vi "_CSMOFGV Dequeue.vi"(8 "Error In":errorcluster caption="error in (no error)", 9 "Dequeue Timeout (0ms)":i32, 10 "State (S) In (\"\")":string, 11 "CSMQ In":T1={"info"={"Module Name"="", "Requested Name"="", "Group Name"="", "Mode"=enum."Stand Alone", "Allowed Messages"=[]}, "Refs"={"WatchDogQ"=refnum, "CSMDataDVR"=refnum, "Queue"={"HPriorityQ"=refnum, "LowPriorityQ"=refnum}, "GroupDataDVR"=refnum, "TagMap"=refnum, "ExitEvent"=refnum, "NewStateEvent"=refnum, "StatusEvent"=refnum, "InterruptEvent"=refnum}}) -> (0 "error out":errorcluster, 2 "States Out":string, 3 "CSMQ Out":T1={"info"={"Module Name"="", "Requested Name"="", "Group Name"="", "Mode"=enum."Stand Alone", "Allowed Messages"=[]}, "Refs"={"WatchDogQ"=refnum, "CSMDataDVR"=refnum, "Queue"={"HPriorityQ"=refnum, "LowPriorityQ"=refnum}, "GroupDataDVR"=refnum, "TagMap"=refnum, "ExitEvent"=refnum, "NewStateEvent"=refnum, "StatusEvent"=refnum, "InterruptEvent"=refnum}})   [LabVIEW 2017, in "Communicable State Machine.lvlib"]
uses:
  Communicable State Machine.lvlib
  _CSMObj.ctl
  _CSMObj-Info.ctl
  Typedef/_CSM_MODE.ctl
  _CSMObj-Refs.ctl
  _CSMObj-Data.ctl
  Typedef/_CSM_MSG_TYPE.ctl
  Priority Queue/Priority Queue.ctl
  Typedef/_Cross CSM State Data.ctl
  Typedef/_Cross CSM State Response.ctl
  Typedef/_CSM_Response Source Message.ctl
  Priority Queue/def-Data(LowPRI-Q).ctl
  _CSMObj-ModeData.ctl
  Typedef/_CSM Status Change Event Data.ctl
  AdvanceAPI/CSM - Make String Arguments Safe.vi
  AdvanceAPI/CSM - Keywords.vi
  _Shared/CSM Shared.lvlib
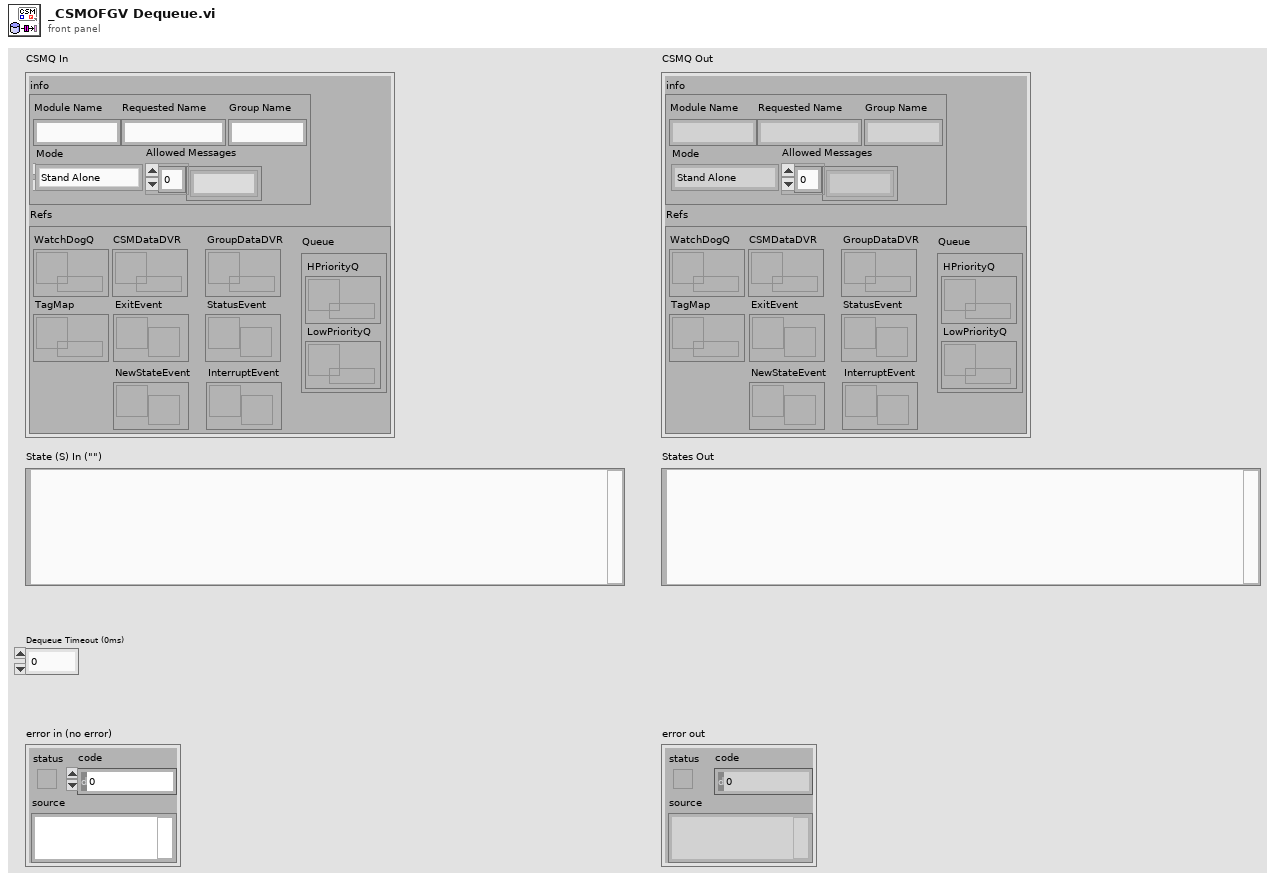
[diagram p1: front panel]
types:
  T1 = typedef "Communicable State Machine.lvlib/_CSMObj.ctl" = cluster{"info":T2, "Refs":T4}
  T2 = typedef "Communicable State Machine.lvlib/_CSMObj-Info.ctl" = cluster{"Module Name":string, "Requested Name":string, "Group Name":string, "Mode":T3, "Allowed Messages":string[]}
  T3 = typedef "Communicable State Machine.lvlib/_CSM_MODE.ctl" = enum16{"Not Exist", "Stand Alone", "CSM", "Worker", "Worker Agent", "Chain Node", "Chain"}
  T4 = typedef "Communicable State Machine.lvlib/_CSMObj-Refs.ctl" = cluster{"WatchDogQ":refnum<queue>, "CSMDataDVR":refnum<data-value>, "Queue":T5, "GroupDataDVR":refnum<data-value>, "TagMap":refnum<data-value>, "ExitEvent":refnum<user-event>, "NewStateEvent":refnum<user-event>, "StatusEvent":refnum<user-event>, "InterruptEvent":refnum<user-event>}
  T5 = typedef "Communicable State Machine.lvlib/Priority Queue.ctl" = cluster{"HPriorityQ":refnum<queue>, "LowPriorityQ":refnum<queue>}
  T6 = typedef "Communicable State Machine.lvlib/_CSM_MSG_TYPE.ctl" = enum16{"Sync Message(-@)", "Async Message(->)", "Async without Response(->|)", "Async Response", "Broadcast(-><all>)", "Broadcast(-><status>)", "Broadcast(-><interrupt>)", "Append to JKISM States", "Append to JKISM States(High Priority)", "Broadcast(-><state>)", "<None>"}
  T7 = typedef "Communicable State Machine.lvlib/_CSMObj-Data.ctl" = cluster{"RemoteMessge?":bool, "error":errorcluster, "Return State":string, "Initialized":enum16{"Initializing", "Ready", "Exiting"}, "InternalRegistryRules":string[], "Return Msg Type":T6, "Current State":string, "Remaing JKISM Queue":string}
  T8 = typedef "Communicable State Machine.lvlib/_Cross CSM State Data.ctl" = cluster{"Msg Type":T6, "state":string, "args":string, "source":string, "RespQ":refnum<queue>, "Response For Message":T9, "Target":string}
  T9 = typedef "Communicable State Machine.lvlib/_CSM_Response Source Message.ctl" = cluster{"‘State":string, "’Arguments":string, "’Error":errorcluster}
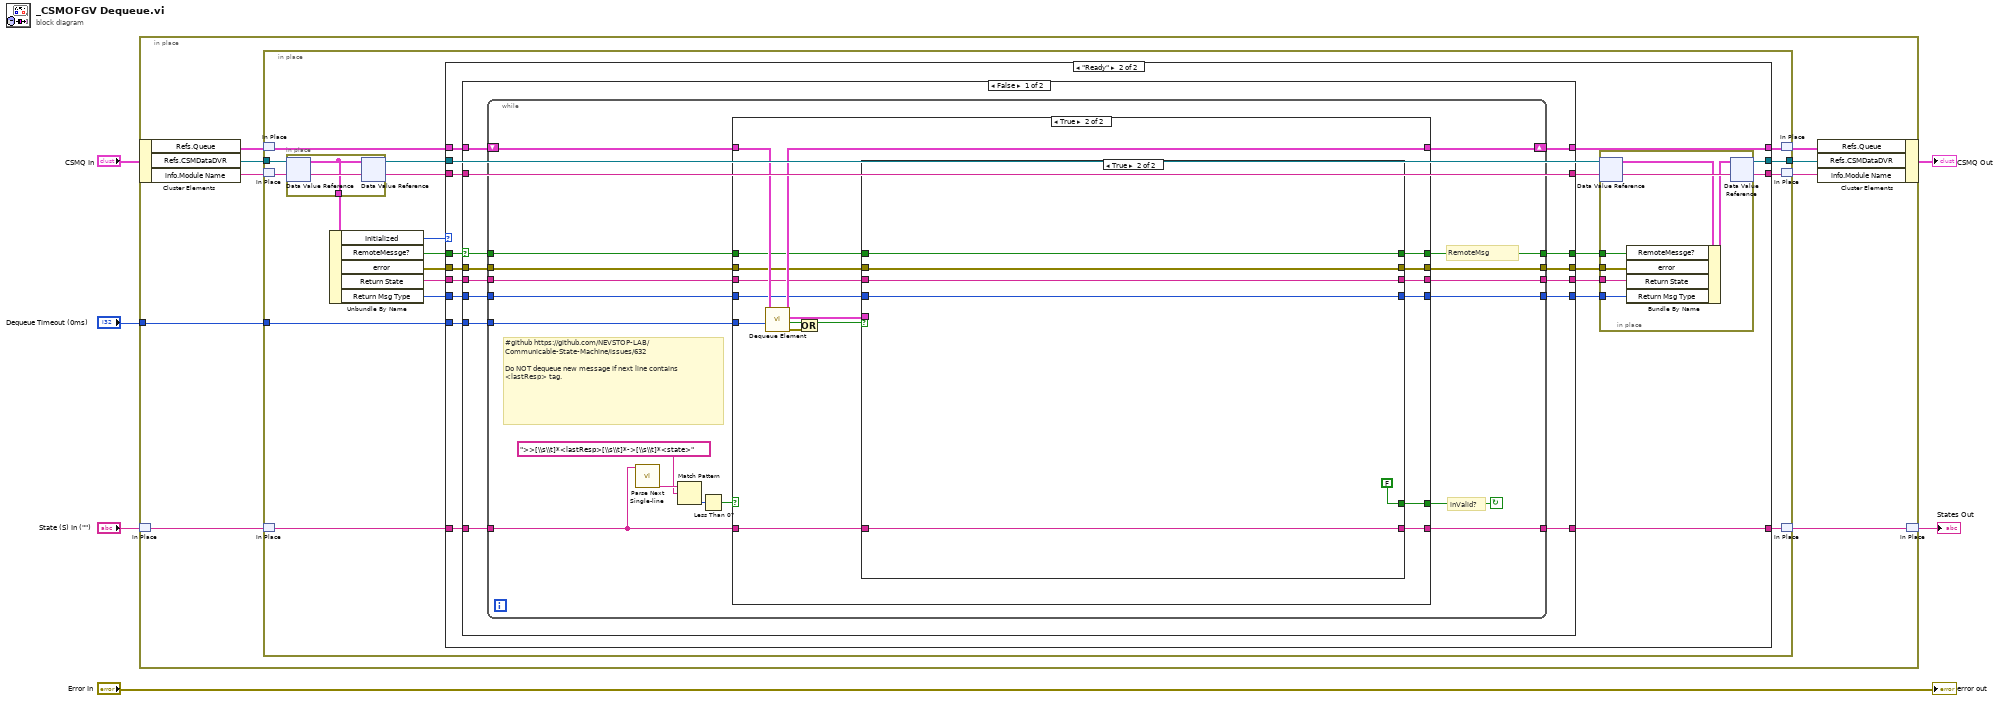
[diagram p0: block diagram]
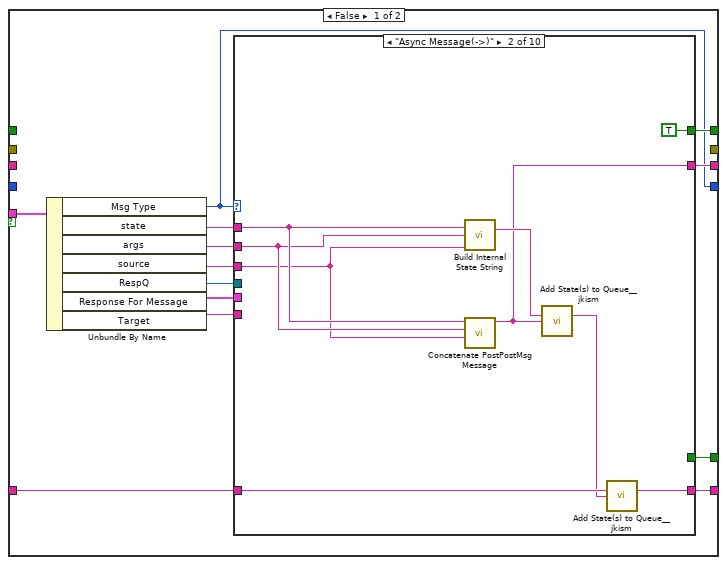
[diagram p4: hidden frame]
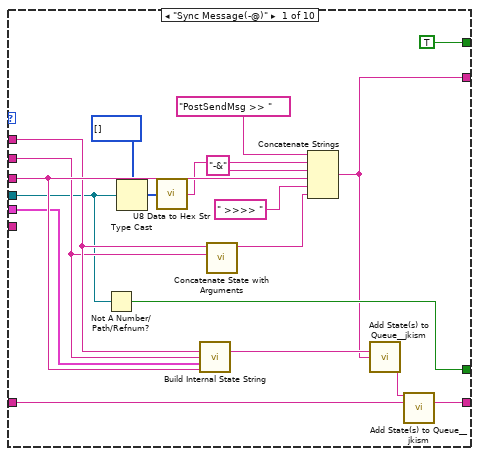
[diagram p5: hidden frame]
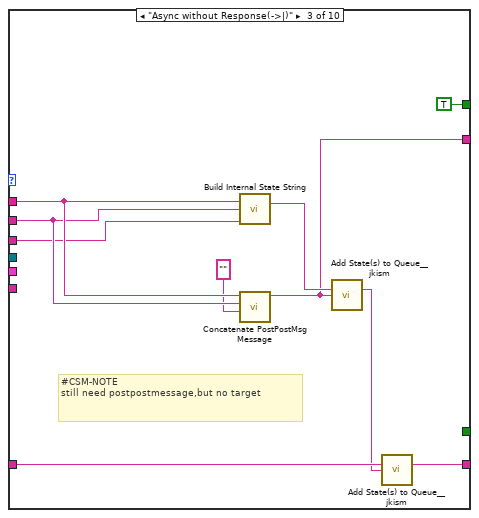
[diagram p6: hidden frame]
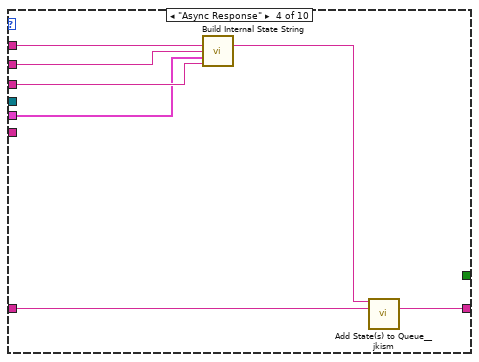
[diagram p7: hidden frame]
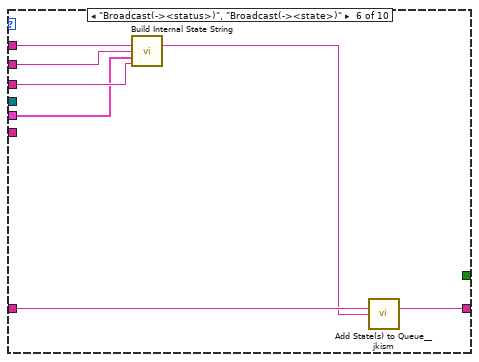
[diagram p9: hidden frame]
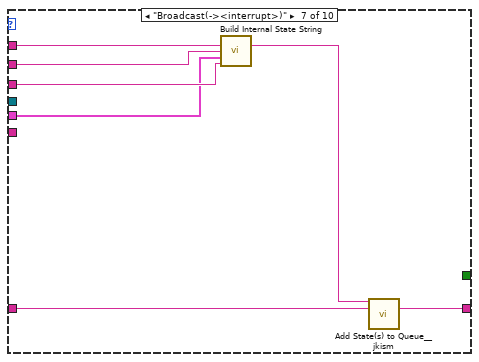
[diagram p10: hidden frame]
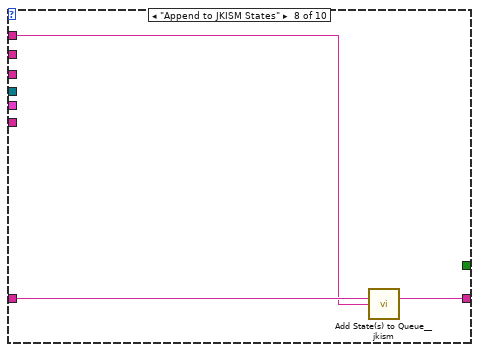
[diagram p11: hidden frame]
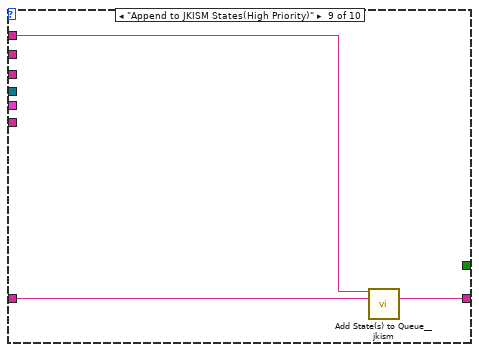
[diagram p12: hidden frame]
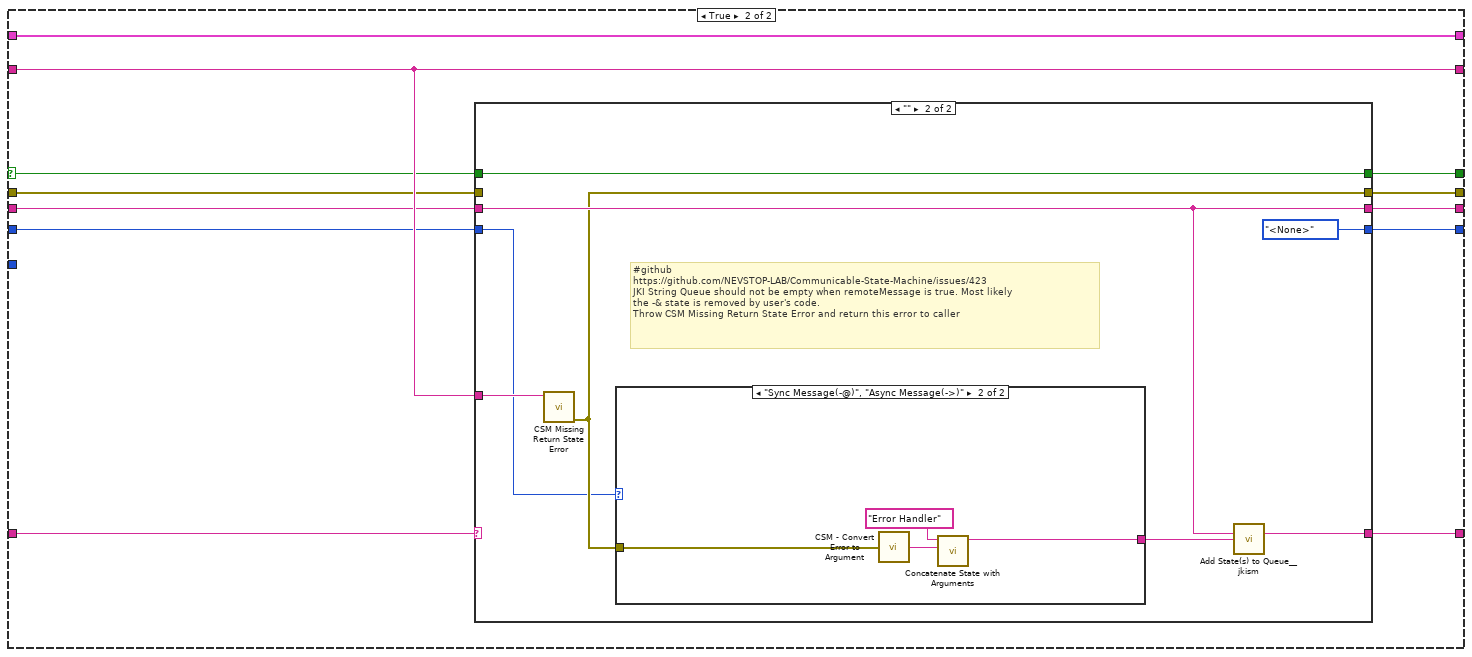
[diagram p14: hidden frame]
diagram:
  n1 = in-place "In Place Element Structure" {
    in-place-border: "Dequeue Timeout (0ms)" -> [w13]
    n2 = in-place-cluster #1("CSMQ In") -> ("Refs.Queue"=w15:T5, "Refs.CSMDataDVR"=w10:refnum<data-value>, "info.Module Name"=w7:string)
    n3 = in-place-match #2("State (S) In (\"\")") -> (w12:string)
    n4 = in-place {
      in-place-border: w13 -> [w29]
      in-place-border: w10 -> [w26]
      in-place-border: [w23] -> w9
      n5 = in-place-match #3(w15) -> (w30:T5)
      n6 = in-place-match #4(w7) -> (w19:string)
      n7 = in-place-match #5(w12) -> (w28:string)
      n8 = in-place {
        in-place-border: [w230] -> w25
        n9 = in-place-dvr #6(w26) -> (w230:T7)  [unwired: 1 out]
        n10 = in-place-dvr #6(w230) -> (w24:refnum<data-value>)  [unwired: 1 out]
      }
      n11 = Unbundle By Name(w25) -> ("Initialized"=w17:enum16{"Initializing", "Ready", "Exiting"}, "RemoteMessge?"=w22:bool, "error"=w21:errorcluster, "Return State"=w20:string, "Return Msg Type"=w16:T6)
      n12 = case shown="\"Ready\"" w17 {
        tunnel: [w35 w52] -> w31
        tunnel: w30 -> [w35 w51]
        tunnel: w29 -> [_ w50]
        tunnel: w28 -> [w32 w49]
        tunnel: [w32 w48] -> w27
        tunnel: w24 -> [w34 w47]
        tunnel: [w34 w46] -> w23
        tunnel: w22 -> [_ w44]
        tunnel: w21 -> [_ w42]
        tunnel: w20 -> [_ w40]
        tunnel: w19 -> [w33 w39]
        tunnel: [w33 w38] -> w18
        tunnel: w16 -> [_ w36]
        frame "Initializing", "Exiting", Default {
        }
        frame "Ready" {
          n13 = case shown="False" w44 {
            selector: w44 -> [w66 w203]
            tunnel: [w71 w212] -> w52
            tunnel: w51 -> [w72 w212]
            tunnel: w50 -> [w70 _]
            tunnel: w49 -> [w69 w206]
            tunnel: [w68 w205] -> w48
            tunnel: [w67 w204] -> w45
            tunnel: [w65 w210] -> w43
            tunnel: w42 -> [w64 w209]
            tunnel: [w63 w208] -> w41
            tunnel: w40 -> [w62 w207]
            tunnel: w39 -> [w61 w211]
            tunnel: [w61 w211] -> w38
            tunnel: [w60 w202] -> w37
            tunnel: w36 -> [w59 w201]
            frame False {
              n14 = while {
                tunnel: w70 -> [w88]
                shift-right: [w89] -> w71
                shift-left: w72 -> [w90]
                tunnel: w66 -> [w85]
                tunnel: [w86] -> w67
                tunnel: w69 -> [w77]
                tunnel: [w87] -> w68
                tunnel: [w83] -> w65
                tunnel: w64 -> [w82]
                tunnel: [w81] -> w63
                tunnel: w62 -> [w80]
                tunnel: [w79] -> w60
                tunnel: w59 -> [w78]
                stop <- w84 continue-if-true
                # "#github https://github.com/NEVSTOP-LAB/Communicable-State-Machine/issues/632\n\nDo NOT dequeue new message if next line contains <lastResp> tag."
                # "inValid?"
                # "RemoteMsg"
                n15 = call "Parse Next Single-line.vi"("States Queue"=w77) -> ("Next Single-line State"=w76:string)  [unwired: 9 in, 1 out]
                n16 = Match Pattern(string=w76, regular expression=">>[\\s\\t]*<lastResp>[\\s\\t]*->[\\s\\t]*<state>" ("string")) -> (offset past match=w75:i32)  [unwired: 1 in, 3 out]
                n17 = Less Than 0?(x=w75) -> (x < 0?=w74:bool)
                n18 = case shown="True" w74 {
                  tunnel: w90 -> [w96 w114]
                  tunnel: [w96 w113] -> w89
                  tunnel: w88 -> [_ w112]
                  tunnel: w77 -> [w91 w110]
                  tunnel: [w91 w109] -> w87
                  tunnel: [w94 w105] -> w86
                  tunnel: w85 -> [w94 w104]
                  tunnel: [_ w103] -> w84
                  tunnel: [w95 w102] -> w83
                  tunnel: w82 -> [w95 w101]
                  tunnel: [w93 w100] -> w81
                  tunnel: w80 -> [w93 w99]
                  tunnel: [w92 w98] -> w79
                  tunnel: w78 -> [w92 w97]
                  frame False {
                  }
                  frame True {
                    n19 = call "Dequeue Element.vi"("Timeout In ms (-1)"=w112, "Priority Queue"=w114) -> ("error out"=w106:errorcluster, "Timed Out?"=w107:bool, "Cross JKI State Machine State"=w111:T8, "Priority Queue (Dup)"=w113:T5)  [unwired: 5 in, 1 out]
                    n20 = Or(x=w107, y=w106) -> (x .or. y?=w108:bool)
                    n21 = case shown="True" w108 {
                      tunnel: w110 -> [w127 w200]
                      tunnel: [w126 w200] -> w109
                      tunnel: w111 -> [w121 _]
                      tunnel: [w118 w199] -> w105
                      tunnel: w104 -> [_ w199]
                      tunnel: [w117 FALSE] -> w103
                      tunnel: [_ w197] -> w102
                      tunnel: w101 -> [_ w197]
                      tunnel: [w116 w196] -> w100
                      tunnel: w99 -> [_ w196]
                      tunnel: [w115 w195] -> w98
                      tunnel: w97 -> [_ w195]
                      frame False {
                        n22 = Unbundle By Name(w121) -> ("Msg Type"=w115:T6, "state"=w124:string, "args"=w123:string, "source"=w122:string, "RespQ"=w125:refnum<queue>, "Response For Message"=w120:T9, "Target"=w119:string)
                        n23 = case shown="\"Async Message(->)\"" w115 {
                          tunnel: w127 -> [w146 w155 w165 w172 w173 w180 w187 w190 w193 w194]
                          tunnel: [w145 w154 w164 w171 w173 w179 w186 w189 w192 w194] -> w126
                          tunnel: w125 -> [w130 _ _ _ _ _ _ _ _ _]
                          tunnel: w124 -> [w136 w150 w160 w168 _ w176 w183 w188 w191 _]
                          tunnel: w123 -> [w135 w149 w159 w170 _ w178 w185 _ _ _]
                          tunnel: w122 -> [w139 w148 w158 w169 _ w177 w184 _ _ _]
                          tunnel: w120 -> [w137 _ _ w166 _ w175 w182 _ _ _]
                          tunnel: w119 -> [_ _ _ _ _ _ _ _ _ _]
                          tunnel: [TRUE TRUE TRUE _ _ _ _ _ _ _] -> w118
                          tunnel: [w129 _ _ _ _ _ _ _ _ _] -> w117
                          tunnel: [w128 w147 w156 _ _ _ _ _ _ _] -> w116
                          frame "Sync Message(-@)" {
                            n24 = Not A Number/Path/Refnum?(number/path/refnum=w130) -> (NaN/Path/Refnum?=w129:bool)
                            n25 = Type Cast(type=u8[] [], x=w130) -> (*(type *) &x=w132:u8[])
                            n26 = call "U8 Data to Hex Str.vi"("U8 Data[]"=w132) -> ("HEX String (0-9,A-F)"=w131:string)
                            n27 = call "Build Internal State String.vi"("State"=w136, "Arguments (\"\")"=w135, "Additional Information"=w137, "Source (\"\")"=w139) -> ("State With Arguments"=w142:string)  [unwired: 11 in]
                            n28 = call "Concatenate State with Arguments.vi"("Arguments"=w135, "State"=w136) -> ("State With Arguements"=w134:string)  [unwired: 9 in]
                            n29 = Concatenate Strings("PostSendMsg >> " ("State(s) at Back (\"\")"), w131, "-&" ("string"), w139, " >>>> " ("string"), w134) -> (w128:string)
                            n30 = call "Add State(s) to Queue__jkism.vi"("State(s) in (\"\")"=w142, "State(s) at Back (\"\")"=w128) -> ("States Out"=w144:string)  [unwired: 13 in]
                            n31 = call "Add State(s) to Queue__jkism.vi"("State(s) in Front (\"\")"=w144, "State(s) in (\"\")"=w146) -> ("States Out"=w145:string)  [unwired: 13 in]
                          }
                          frame "Async Message(->)" {
                            n32 = call "Build Internal State String.vi"("State"=w150, "Arguments (\"\")"=w149, "Source (\"\")"=w148) -> ("State With Arguments"=w153:string)  [unwired: 12 in]
                            n33 = call "Concatenate PostPostMsg Message.vi"("Source"=w148, "Arguments"=w149, "Async-Message"=w150) -> ("PostPostMsg Message"=w147:string)  [unwired: 8 in]
                            n34 = call "Add State(s) to Queue__jkism.vi"("State(s) in (\"\")"=w153, "State(s) at Back (\"\")"=w147) -> ("States Out"=w151:string)  [unwired: 13 in]
                            n35 = call "Add State(s) to Queue__jkism.vi"("State(s) in (\"\")"=w155, "State(s) at Back (\"\")"=w151) -> ("States Out"=w154:string)  [unwired: 13 in]
                          }
                          frame "Async without Response(->|)" {
                            # "#CSM-NOTE\nstill need postpostmessage,but no target"
                            n36 = call "Build Internal State String.vi"("State"=w160, "Arguments (\"\")"=w159, "Source (\"\")"=w158) -> ("State With Arguments"=w163:string)  [unwired: 12 in]
                            n37 = call "Concatenate PostPostMsg Message.vi"("Source"="", "Arguments"=w159, "Async-Message"=w160) -> ("PostPostMsg Message"=w156:string)  [unwired: 8 in]
                            n38 = call "Add State(s) to Queue__jkism.vi"("State(s) in (\"\")"=w163, "State(s) at Back (\"\")"=w156) -> ("States Out"=w161:string)  [unwired: 13 in]
                            n39 = call "Add State(s) to Queue__jkism.vi"("State(s) in (\"\")"=w165, "State(s) at Back (\"\")"=w161) -> ("States Out"=w164:string)  [unwired: 13 in]
                          }
                          frame "Async Response" {
                            n40 = call "Build Internal State String.vi"("State"=w168, "Arguments (\"\")"=w170, "Additional Information"=w166, "Source (\"\")"=w169) -> ("State With Arguments"=w167:string)  [unwired: 11 in]
                            n41 = call "Add State(s) to Queue__jkism.vi"("State(s) in Front (\"\")"=w167, "State(s) in (\"\")"=w172) -> ("States Out"=w171:string)  [unwired: 13 in]
                          }
                          frame "Broadcast(-><all>)" {
                            # "#CSM-NOTE\nshould no be here"
                          }
                          frame "Broadcast(-><status>)", "Broadcast(-><state>)" {
                            n42 = call "Build Internal State String.vi"("State"=w176, "Arguments (\"\")"=w178, "Additional Information"=w175, "Source (\"\")"=w177) -> ("State With Arguments"=w174:string)  [unwired: 11 in]
                            n43 = call "Add State(s) to Queue__jkism.vi"("State(s) in (\"\")"=w180, "State(s) at Back (\"\")"=w174) -> ("States Out"=w179:string)  [unwired: 13 in]
                          }
                          frame "Broadcast(-><interrupt>)" {
                            n44 = call "Build Internal State String.vi"("State"=w183, "Arguments (\"\")"=w185, "Additional Information"=w182, "Source (\"\")"=w184) -> ("State With Arguments"=w181:string)  [unwired: 11 in]
                            n45 = call "Add State(s) to Queue__jkism.vi"("State(s) in Front (\"\")"=w181, "State(s) in (\"\")"=w187) -> ("States Out"=w186:string)  [unwired: 13 in]
                          }
                          frame "Append to JKISM States" {
                            n46 = call "Add State(s) to Queue__jkism.vi"("State(s) in (\"\")"=w190, "State(s) at Back (\"\")"=w188) -> ("States Out"=w189:string)  [unwired: 13 in]
                          }
                          frame "Append to JKISM States(High Priority)" {
                            n47 = call "Add State(s) to Queue__jkism.vi"("State(s) in Front (\"\")"=w191, "State(s) in (\"\")"=w193) -> ("States Out"=w192:string)  [unwired: 13 in]
                          }
                          frame "<None>" {
                          }
                        }
                      }
                      frame True {
                      }
                    }
                  }
                }
              }
            }
            frame True {
              n48 = case shown="\"\"" w206 {
                selector: w206 -> [w215 _]
                tunnel: w211 -> [_ w225]
                tunnel: [w217 w222] -> w210
                tunnel: w209 -> [w217 _]
                tunnel: [w216 w223] -> w208
                tunnel: w207 -> [w216 w223]
                tunnel: [w215 w224] -> w205
                tunnel: [w214 w219] -> w204
                tunnel: w203 -> [w214 w219]
                tunnel: [w213 _CSM_MSG_TYPE."<None>" ("Return Msg Type")] -> w202
                tunnel: w201 -> [w213 w218]
                frame Default {
                }
                frame "" {
                  # "#github \nhttps://github.com/NEVSTOP-LAB/Communicable-State-Machine/issues/423\nJKI String Queue should not be empty when remoteMessage is true. Most likely\nthe -& state is removed by user's code. \nThrow CSM Missing Return State Error and return this error to caller"
                  n49 = call "CSM Missing Return State Error.vi"("Arguments (As CSM Name)"=w225) -> ("error out"=w222:errorcluster)  [unwired: 10 in]
                  n50 = case shown="\"Sync Message(-@)\", \"Async Message(->)\"" w218 {
                    tunnel: w222 -> [_ w229]
                    tunnel: [_ w228] -> w220
                    frame "Async without Response(->|)", Default {
                    }
                    frame "Sync Message(-@)", "Async Message(->)" {
                      n51 = call "CSM - Convert Error to Argument.vi"("Error"=w229) -> ("Argument"=w227:string)  [unwired: 4 in]
                      n52 = call "Concatenate State with Arguments.vi"("Arguments"=w227, "State"="Error Handler") -> ("State With Arguements"=w228:string)  [unwired: 9 in]
                    }
                  }
                  n53 = call "Add State(s) to Queue__jkism.vi"("State(s) in (\"\")"=w223, "State(s) at Back (\"\")"=w220) -> ("States Out"=w224:string)  [unwired: 13 in]
                }
              }
            }
          }
          n54 = in-place {
            in-place-border: w45 -> [w56]
            in-place-border: w43 -> [w55]
            in-place-border: w41 -> [w54]
            in-place-border: w37 -> [w53]
            n55 = in-place-dvr #7(w47) -> (w58:T7)  [unwired: 1 out]
            n56 = Bundle By Name(cluster=w58, "RemoteMessge?"=w56, "error"=w55, "Return State"=w54, "Return Msg Type"=w53) -> (w57:T7)
            n57 = in-place-dvr #7(w57) -> (w46:refnum<data-value>)  [unwired: 1 out]
          }
        }
      }
      n58 = in-place-match #3(w31) -> (w14:T5)
      n59 = in-place-match #4(w18) -> (w8:string)
      n60 = in-place-match #5(w27) -> (w11:string)
    }
    n61 = in-place-cluster #1("Refs.Queue"=w14, "Refs.CSMDataDVR"=w9, "info.Module Name"=w8) -> (→"CSMQ Out":T1)
    n62 = in-place-match #2(w11) -> (→"States Out":string)
  }
  "error out" <- "Error In"
